vi "PosCtrl_Execute.vi"(5 "PosCtrl_Config_Params":T1={"Slope"=0.0, "Offset"=0.0, "Error Deadband"=0.0, "At Reference Count"=13, "Negate Output"=FALSE, "Max Allowd Position"=9e+30, "Min Allowd Position"=-9e+30, "Kd"=0.0, "FilterDerivative"=FALSE}, 6 "Pass_Through_Time":dbl=-1.0 format="%33.4f", 7 "MaxOutput":dbl, 8 "Rev Limit Switch":bool, 9 "Fwd Limit Switch":bool, 10 "CurrentPosition":dbl, 11 "TargetPosition":dbl) -> (1 "OnTarget":bool, 2 "PositionError":dbl, 3 "Output":dbl)   [LabVIEW 2019, in "Trajectory_Library.lvlib"]
doc: "This VI calculates closed loop position control output (CO), provided the Setpoint (SP), and Process Variable (PV). It incorporates a position deadband. It also incorporates output slowdown as the desired position is approached."
uses:
  Trajectory_Library.lvlib
  TypeDef/PosCtrl_Tuning_Type.ctl
  Util_GetTime_U32.vi
  Util_GetTime_U64.vi
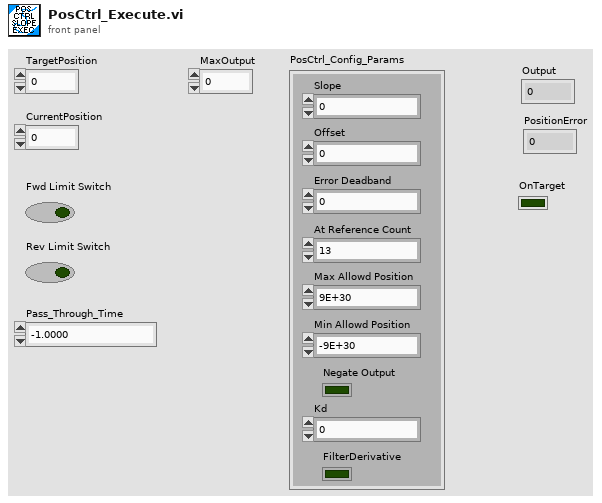
[diagram p1: front panel]
types:
  T1 = typedef "Trajectory_Library.lvlib/PosCtrl_Tuning_Type.ctl" = cluster{"Slope":dbl, "Offset":dbl, "Error Deadband":dbl, "At Reference Count":i32, "Negate Output":bool, "Max Allowd Position":dbl, "Min Allowd Position":dbl, "Kd":dbl, "FilterDerivative":bool}
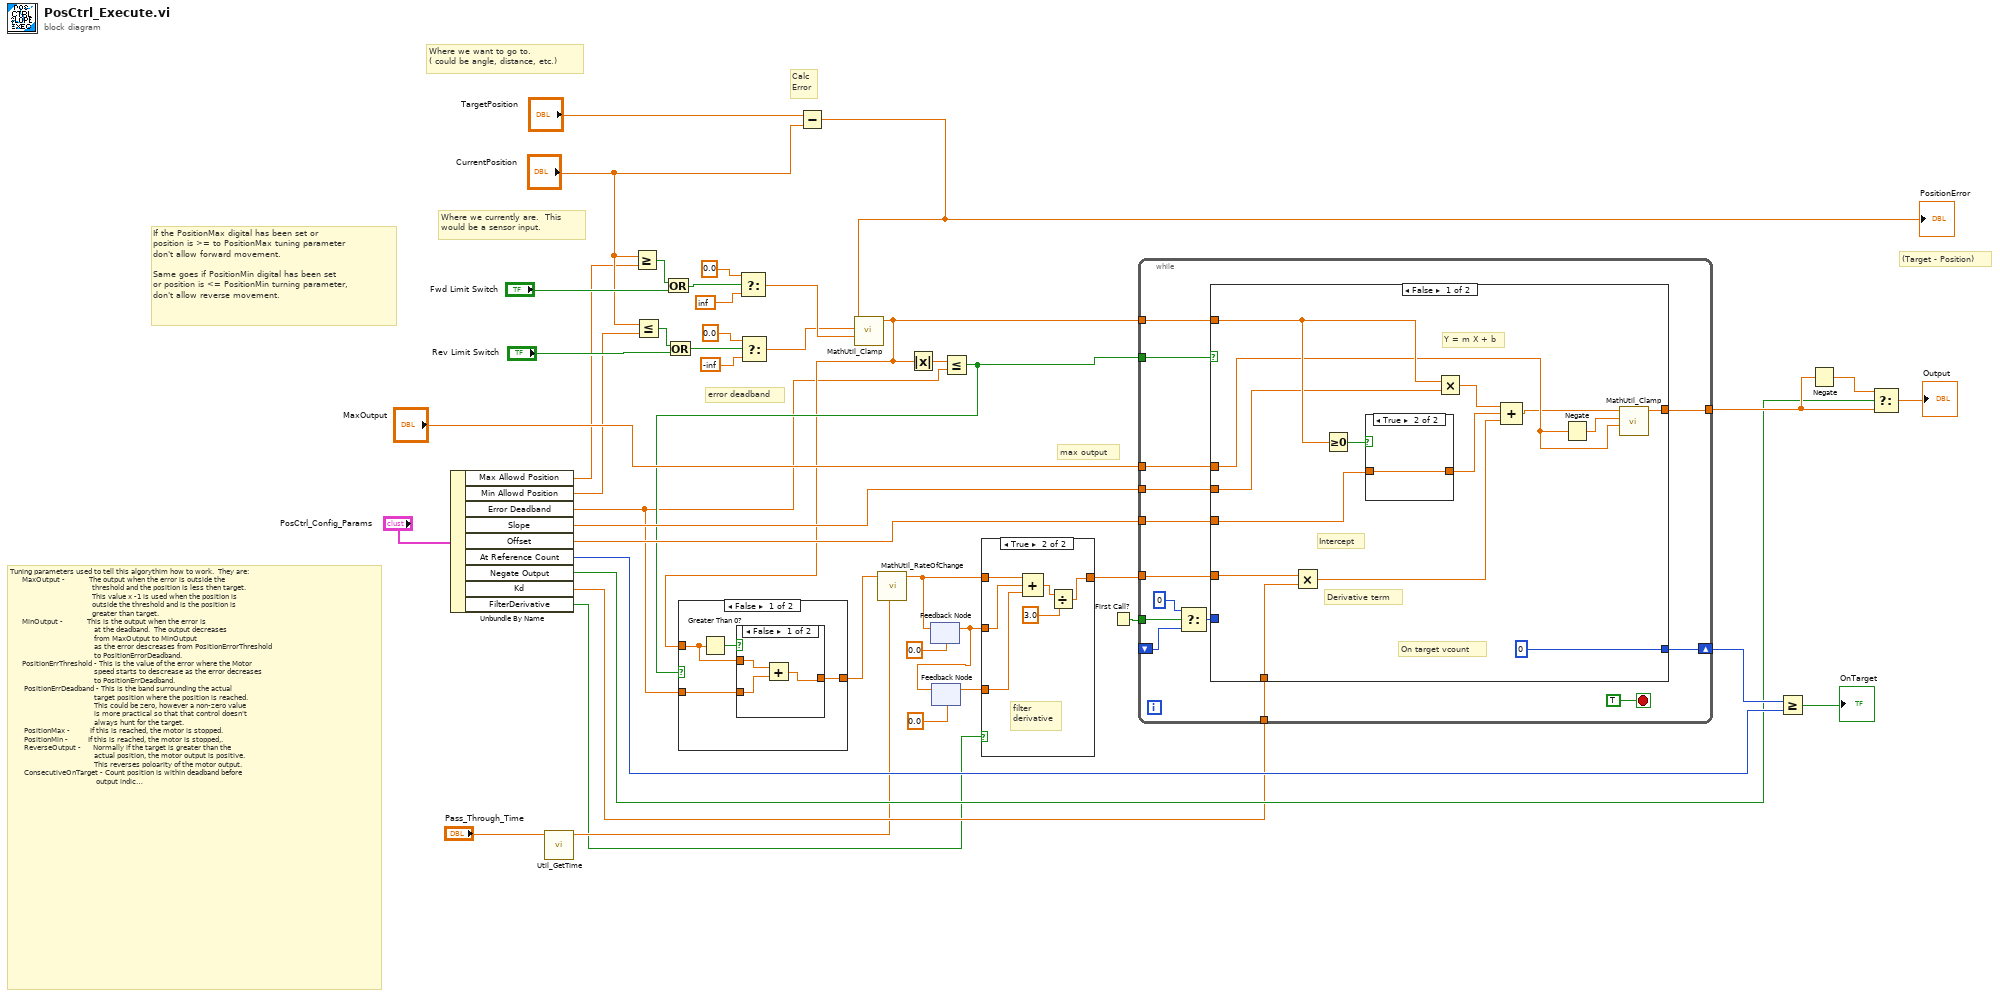
[diagram p0: block diagram]
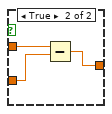
[diagram p3: hidden frame]
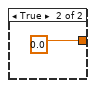
[diagram p4: hidden frame]
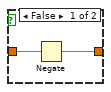
[diagram p5: hidden frame]
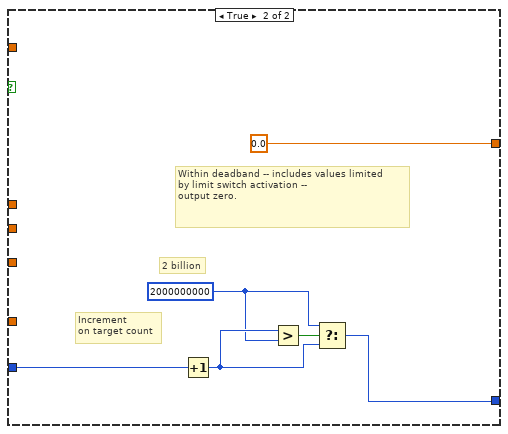
[diagram p6: hidden frame]
diagram:
  # "error deadband"
  # "max output"
  # "(Target - Position)"
  # "Calc\nError"
  # "If the PositionMax digital has been set or\nposition is >= to PositionMax tuning parameter\ndon't allow forward movement.\n\nSame goes if PositionMin digital has been set\nor position is <= PositionMin turning parameter, \ndon't allow reverse movement."
  # "Tuning parameters used to tell this algorythim how to work.  They are:\n      MaxOutput -            The output when the error is outside the \n                                         threshold and the position is less then target.\n                                         This value x -1 is used when the position is\n                                         outside the threshold and is the position is\n                                         greater than target.\n      MinOutput -            This is the output when the error is\n                                          at the deadband.  The output decreases\n                                          from MaxOutput to MinOutput\n                                          as the error descreases from PositionErrorThreshold\n                                          to PositionErrorDeadband.\n      PositionErrThreshold - This is the value of the error where the Motor\n                                          speed starts to descrease as the error decreases\n                                          to PositionErrDeadband.\n       PositionErrDeadband - This is the band surrounding the actual \n                                          target position where the position is reached.\n                                          This could be zero, however a non-zero value\n                                          is more practical so that that control doesn't\n                                          always hunt for the target.\n       PositionMax -          If this is reached, the motor is stopped.\n       PositionMin -          If this is reached, the motor is stopped,.\n       ReverseOutput -      Normally if the target is greater than the \n                                          actual position, the motor output is positive.\n                                          This reverses poloarity of the motor output.\n       ConsecutiveOnTarget - Count position is within deadband before\n                                           output indicates position goal has been\n                                           reached."
  # "Where we currently are.  This \nwould be a sensor input."
  # "Where we want to go to.\n( could be angle, distance, etc.)"
  n1 = Unbundle By Name("PosCtrl_Config_Params") -> ("Max Allowd Position"=w25:dbl, "Min Allowd Position"=w24:dbl, "Error Deadband"=w8:dbl, "Slope"=w34:dbl, "Offset"=w33:dbl, "At Reference Count"=w23:i32, "Negate Output"=w16:bool, "Kd"=w14:dbl, "FilterDerivative"=w1:bool)
  n2 = call "Util_GetTime.vi"("Pass_Through_Time"="Pass_Through_Time") -> ("FPGA_Time_Seconds"=w13:dbl)  [unwired: 8 in, 2 out]
  n3 = Greater Or Equal?(x="CurrentPosition", y=w25) -> (x >= y?=w27:bool)
  n4 = Less Or Equal?(x="CurrentPosition", y=w24) -> (x <= y?=w28:bool)
  n5 = Or(x=w27, y="Fwd Limit Switch") -> (x .or. y?=w32:bool)
  n6 = Or(x=w28, y="Rev Limit Switch") -> (x .or. y?=w31:bool)
  n7 = Select(t=0.0, s=w32, f=inf) -> (s? t:f=w18:dbl)
  n8 = Select(t=0.0, s=w31, f=-inf) -> (s? t:f=w17:dbl)
  n9 = Subtract(x="TargetPosition", y="CurrentPosition") -> (x-y=w19:dbl)
  "PositionError" <- w19
  n10 = call "MathUtil_Clamp.vi"("High Limit"=w18, "Low Limit"=w17, "Value"=w19) -> ("Result"=w9:dbl)  [unwired: 8 in]
  n11 = Absolute Value(x=w9) -> (abs(x)=w12:dbl)
  n12 = feedback #1(0.0 ("Rate_Of_Change")) -> (w3:dbl)
  n13 = feedback #2(0.0 ("Rate_Of_Change")) -> (w2:dbl)
  n14 = feedback-in #2(w3) -> ()
  n15 = Less Or Equal?(x=w12, y=w8) -> (x <= y?=w11:bool)
  n16 = case shown="False" w11 {
    tunnel: [w45 0.0] -> w10
    tunnel: w9 -> [w47 _]
    tunnel: w8 -> [w46 _]
    frame False {
      n17 = Greater Than 0?(x=w47) -> (x > 0?=w48:bool)
      n18 = case shown="False" w48 {
        tunnel: w47 -> [w51 w54]
        tunnel: w46 -> [w50 w53]
        tunnel: [w49 w52] -> w45
        frame False {
          n19 = Add(x=w51, y=w50) -> (x+y=w49:dbl)
        }
        frame True {
          n20 = Subtract(x=w54, y=w53) -> (x-y=w52:dbl)
        }
      }
    }
    frame True {
    }
  }
  n21 = call "MathUtil_RateOfChange.vi"("FPGA_Time_Seconds"=w13, "Input"=w10) -> ("Rate_Of_Change"=w5:dbl)  [unwired: 9 in]
  n22 = feedback-in #1(w5) -> ()
  n23 = case shown="True" w1 {
    tunnel: w5 -> [w56 w62]
    tunnel: [w56 w59] -> w4
    tunnel: w3 -> [_ w58]
    tunnel: w2 -> [_ w57]
    frame False {
    }
    frame True {
      # "filter\nderivative"
      n24 = Compound Arithmetic op=ADD(w62, w58, w57) -> (w61:dbl)
      n25 = Divide(x=w61, y=3.0) -> (x/y=w59:dbl)
    }
  }
  n26 = First Call?() -> (First Call?: T/F=w39:bool)
  n27 = while {
    tunnel: w9 -> [w74]
    tunnel: [w75] -> w20
    tunnel: "MaxOutput" -> [w73]
    shift-right: [w72] -> w37
    shift-left: _ -> [w70]
    tunnel: w39 -> [w71]
    tunnel: w33 -> [w67]
    tunnel: w34 -> [w66]
    tunnel: w4 -> [w65]
    tunnel: w14 -> [w64]
    tunnel: w11 -> [w63]
    stop <- TRUE stop-if-true
    n28 = Select(t=0, s=w71, f=w70) -> (s? t:f=w69:i32)
    n29 = case shown="False" w63 {
      tunnel: [w80 0.0] -> w75
      tunnel: w74 -> [w90 _]
      tunnel: w73 -> [w82 _]
      tunnel: [0 w95] -> w72
      tunnel: w69 -> [_ w98]
      tunnel: w67 -> [w85 _]
      tunnel: w66 -> [w84 _]
      tunnel: w65 -> [w79 _]
      tunnel: w64 -> [w78 _]
      frame False {
        # "Derivative term"
        # "Y = m X + b"
        # "Intercept"
        # "On target vcount"
        n30 = Multiply(x=w79, y=w78) -> (x*y=w77:dbl)
        n31 = Greater Or Equal To 0?(x=w90) -> (x >= 0?=w88:bool)
        n32 = case shown="True" w88 {
          tunnel: w85 -> [w92 w93]
          tunnel: [w91 w93] -> w86
          frame False {
            n33 = Negate(x=w92) -> (-x=w91:dbl)
          }
          frame True {
          }
        }
        n34 = Multiply(x=w90, y=w84) -> (x*y=w87:dbl)
        n35 = Compound Arithmetic op=ADD(w87, w86, w77) -> (w81:dbl)
        n36 = Negate(x=w82) -> (-x=w83:dbl)
        n37 = call "MathUtil_Clamp.vi"("High Limit"=w82, "Low Limit"=w83, "Value"=w81) -> ("Result"=w80:dbl)  [unwired: 8 in]
      }
      frame True {
        w94 = 2000000000 ("y")
        # "2 billion"
        # "Increment\non target count"
        # "Within deadband -- includes values limited \nby limit switch activation --\noutput zero."
        n38 = Increment(x=w98) -> (x+1=w96:i32)
        n39 = Greater?(x=w96, y=w94) -> (0:w97:bool)
        n40 = Select(t=w94, s=w97, f=w96) -> (s? t:f=w95:i32)
      }
    }
  }
  n41 = Greater Or Equal?(x=w37, y=w23) -> (x >= y?=→"OnTarget":bool)
  n42 = Negate(x=w20) -> (-x=w21:dbl)
  n43 = Select(t=w21, s=w16, f=w20) -> (s? t:f=→"Output":dbl)
